vi "数据校验.vi"(8 "长度":i32=2, 9 "偏移量(0)":i32, 11 "字符串":string) -> (1 "校验字符串":string, 3 "数据字符串":string)   [LabVIEW 2025]
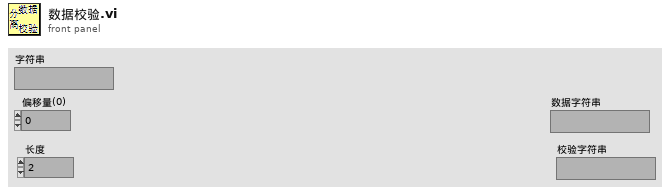
[diagram p1: front panel]
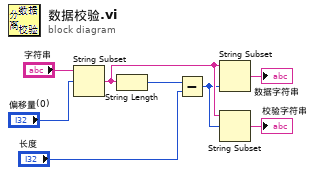
[diagram p0: block diagram]
diagram:
  n1 = String Subset(string="字符串", offset (0)="偏移量(0)") -> (substring=w3:string)  [unwired: 1 in]
  n2 = String Length(string=w3) -> (length=w2:i32)
  n3 = Subtract(x=w2, y="长度") -> (x-y=w1:i32)
  n4 = String Subset(string=w3, length (rest)=w1) -> (substring=→"数据字符串":string)  [unwired: 1 in]
  n5 = String Subset(string=w3, offset (0)=w1) -> (substring=→"校验字符串":string)  [unwired: 1 in]
